vi "core.vi"(8 "H[5] in":u32[](array[numeric]), 11 "W[ ]":u32[](array[numeric])) -> (0 "H[5] out":u32[](array[numeric]))   [LabVIEW 2013, in "SHA-1.lvlib" / "SHA-1.lvclass"]
uses:
  SHA-1.lvclass
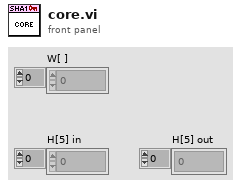
[diagram p1: front panel]
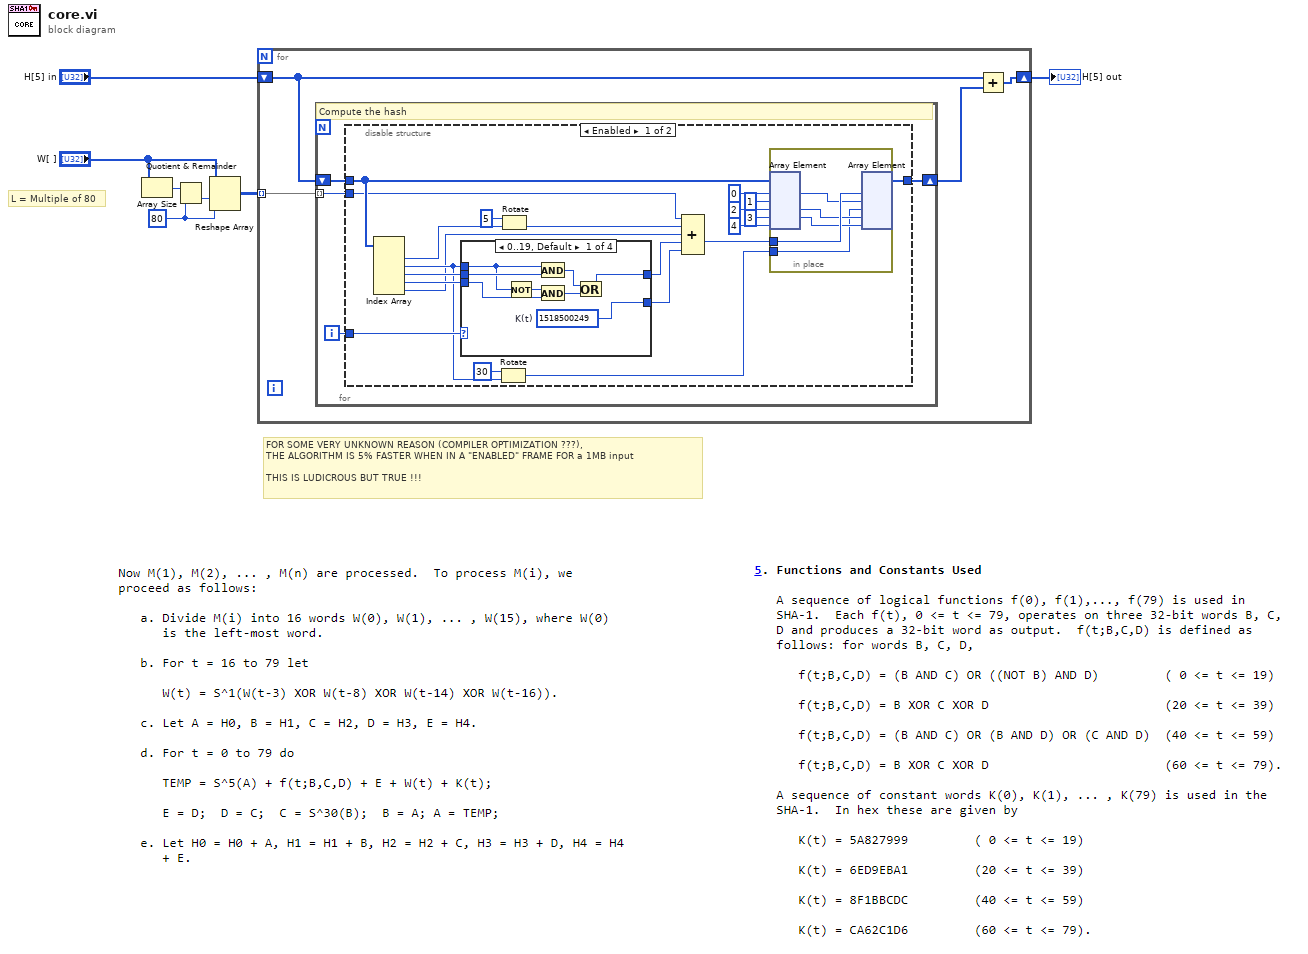
[diagram p0: block diagram]
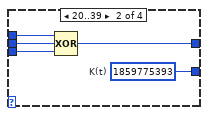
[diagram p2: hidden frame]
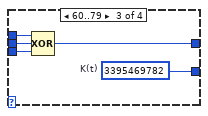
[diagram p3: hidden frame]
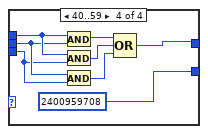
[diagram p4: hidden frame]
diagram:
  w4 = 80 ("y")
  # "FOR SOME VERY UNKNOWN REASON (COMPILER OPTIMIZATION ???), \nTHE ALGORITHM IS 5% FASTER WHEN IN A \"ENABLED\" FRAME FOR a 1MB input\n\nTHIS IS LUDICROUS BUT TRUE !!!"
  # "L = Multiple of 80"
  n1 = Array Size(array="W[ ]") -> (size(s)=w6:i32)
  n2 = Quotient & Remainder(x=w6, y=w4) -> (floor(x/y)=w5:i32)  [unwired: 1 out]
  n3 = Reshape Array("W[ ]", w5, w4) -> (w2:u32[][])
  n4 = for {
    tunnel: w2 -> [w8] mode=indexing
    shift-right: [w10] -> w7
    shift-left: "H[5] in" -> [w11]
    n5 = for {
      shift-right: [w13] -> w9
      shift-left: w11 -> [w14]
      tunnel: w8 -> [w12] mode=indexing
      i -> [w15]
      # "Compute the hash"
      n6 = disable-structure shown="Enabled" {
        disable-tunnel: w15 -> [w36 _]
        disable-tunnel: w14 -> [w30 _]
        disable-tunnel: [w21 _] -> w13
        disable-tunnel: w12 -> [w18 _]
        frame Enabled {
          n7 = Index Array(array=w30) -> (element #1=w16:u32, element #2=w28:u32, element #3=w33:u32, element #4=w32:u32, element #5=w17:u32)  [unwired: 5 in]
          n8 = case shown="0..19, Default" w36 {
            tunnel: w28 -> [w44 w54 w59 w67]
            tunnel: w33 -> [w45 w53 w58 w66]
            tunnel: w32 -> [w46 w52 w57 w65]
            tunnel: [w43 w50 w55 w61] -> w19
            tunnel: [w42 w51 w56 u32 2400959708] -> w20
            frame 0..19, Default {
              w42 = u32 1518500249  # K(t)
              n9 = Not(x=w44) -> (.not. x?=w49:u32)
              n10 = And(x=w44, y=w45) -> (x .and. y?=w47:u32)
              n11 = And(x=w49, y=w46) -> (x .and. y?=w48:u32)
              n12 = Or(x=w47, y=w48) -> (x .or. y?=w43:u32)
            }
            frame 20..39 {
              w51 = u32 1859775393  # K(t)
              n13 = Compound Arithmetic op=XOR(w54, w53, w52) -> (w50:u32)
            }
            frame 60..79 {
              w56 = u32 3395469782  # K(t)
              n14 = Compound Arithmetic op=XOR(w59, w58, w57) -> (w55:u32)
            }
            frame 40..59 {
              n15 = And(x=w67, y=w66) -> (x .and. y?=w64:u32)
              n16 = And(x=w67, y=w65) -> (x .and. y?=w63:u32)
              n17 = And(x=w66, y=w65) -> (x .and. y?=w62:u32)
              n18 = Compound Arithmetic op=OR(w64, w63, w62) -> (w61:u32)
            }
          }
          n19 = Rotate(1:w28, 2:i8 30 ("y")) -> (0:w22:u32)
          n20 = Rotate(1:w16, 2:i8 5 ("y")) -> (0:w34:u32)
          n21 = Compound Arithmetic op=ADD(w18, w34, w17, w19, w20) -> (w31:u32)
          n22 = in-place {
            in-place-border: w31 -> [w41]
            in-place-border: w22 -> [w37]
            n23 = in-place-array #1(w30, 0, 1, 2, 3, 4) -> (w40:u32, w39:u32, w38:u32)  [unwired: 2 out]
            n24 = in-place-array #1(w41, w40, w37, w39, w38) -> (w21:u32[])  [unwired: 5 out]
          }
        }
        frame Disabled {
        }
      }
    }
    n25 = Add(x=w11, y=w9) -> (x+y=w10:u32[])
  }
  "H[5] out" <- w7
